vi "Call VI.vi"(4 "output info":T1[](array[typedef]), 6 "input info":T2[](array[typedef]), 8 "error in (no error)":errorcluster, 9 "Input Values":string[](array[string]), 10 "Input Names":string[](array[string]), 11 "VI in":refnum<vi>) -> (0 "error out":errorcluster, 1 "output values":string[](array[string]), 2 "output names":string[](array[string]), 3 "pictures":string[](array[string]))   [LabVIEW 2020, in "MCP Server.lvlib"]
uses:
  MCP Server.lvlib
  <vilib>/JDP Science/JSONtext/LVClass Serializer/JSONtext LVClass Serializer.lvclass
  e41d13a5-b533-4b14-93c6-4ba0c6d1a2bf.vi
  b3e15f38-d5ce-4610-9e48-04c139622bf1.vi
  b8448edb-b4b5-47d7-90b3-aea56ff88df2.vi
  989a8bd6-30de-4821-a40a-8a1d239f579d.vi
  8b9ff06f-0ef6-44a3-acf4-59db1b6b1b31.vi
  0616d323-15ae-486a-97f1-8f6250f713f5.vi
  9d91f7f2-9bb6-4ecb-af38-d838d0deb514.vi
  fd11c23e-f9de-4047-abc2-5cee66b205fd.vi
  1521ffbb-a9e1-42f7-9593-99dcb95d3f2d.vi
  522b1827-3836-432c-b8b2-8f0c55f6feb7.vi
  4168f984-ecba-4b3e-98aa-6b303e1fc845.vi
  4c506424-2eda-4aef-885b-07ff0af22ab5.vi
  543640a1-fb1b-49d2-854d-672a7e8b1deb.vi
  bf9e786f-d1ab-471f-a68b-f7992835e449.vi
  7e5c8ca1-4dad-4b78-a054-e5ecb6fe69da.vi
  804d9a9c-1e56-403f-8063-8c6c0e8f0982.vi
  Input Parameter.ctl
  Output Parameter.ctl
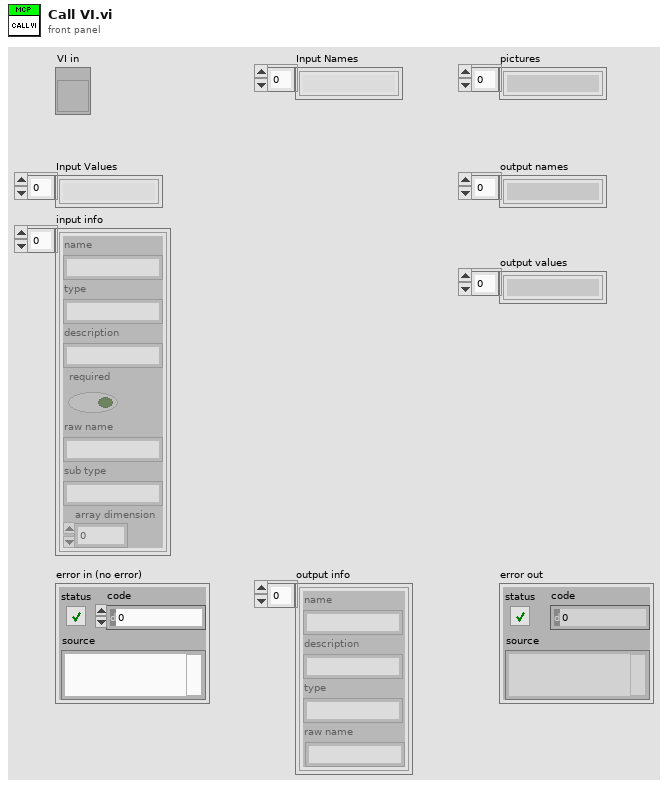
[diagram p1: front panel]
types:
  T1 = typedef "MCP Server.lvlib/Output Parameter.ctl" = cluster{"name":string, "description":string, "type":string, "raw name":string}
  T2 = typedef "MCP Server.lvlib/Input Parameter.ctl" = cluster{"name":string, "type":string, "description":string, "required":bool, "raw name":string, "sub type":string, "array dimension":i32}
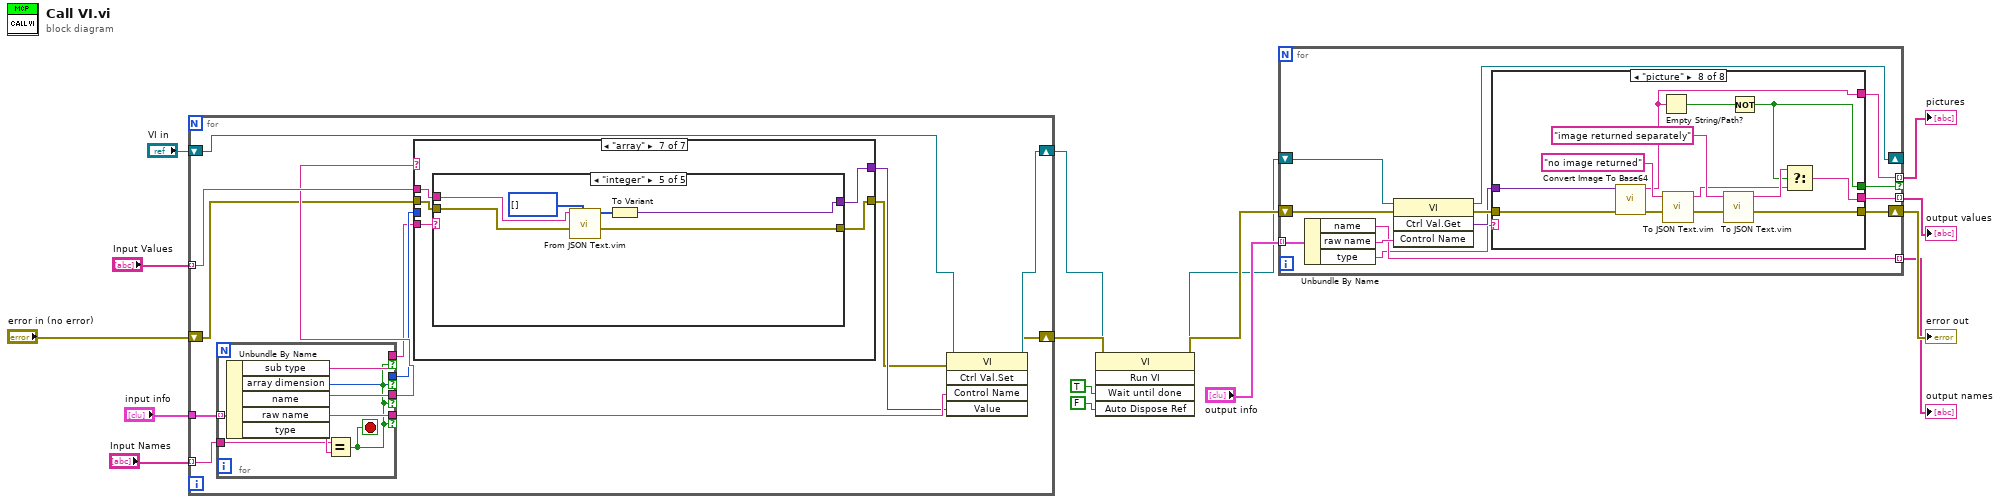
[diagram p0: block diagram]
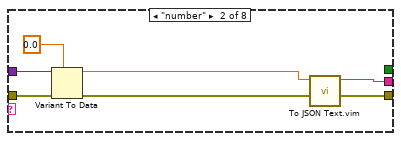
[diagram p3: hidden frame]
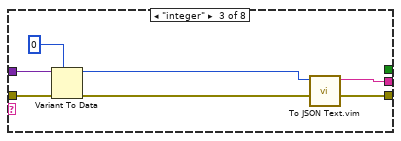
[diagram p4: hidden frame]
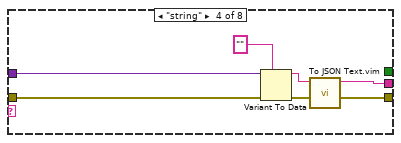
[diagram p5: hidden frame]
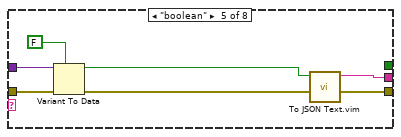
[diagram p6: hidden frame]
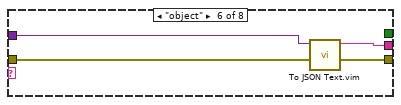
[diagram p7: hidden frame]
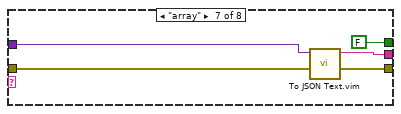
[diagram p8: hidden frame]
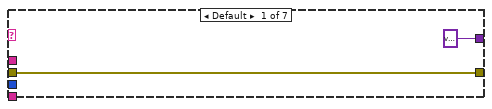
[diagram p9: hidden frame]
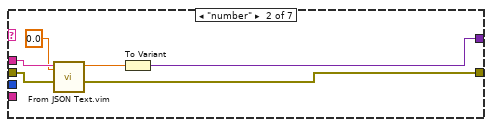
[diagram p10: hidden frame]
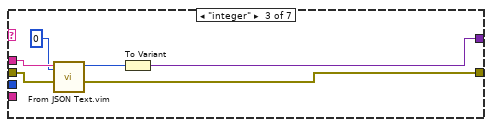
[diagram p11: hidden frame]
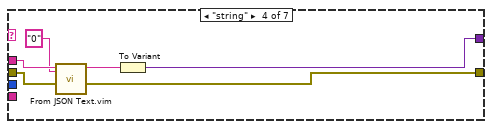
[diagram p12: hidden frame]
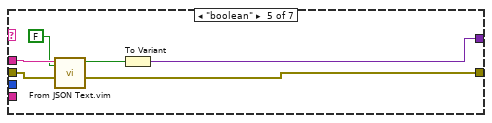
[diagram p13: hidden frame]
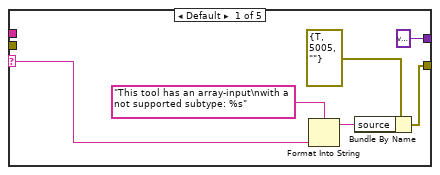
[diagram p15: hidden frame]
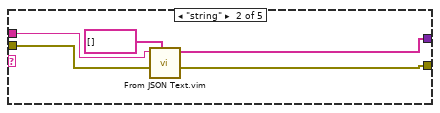
[diagram p16: hidden frame]
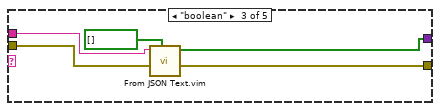
[diagram p17: hidden frame]
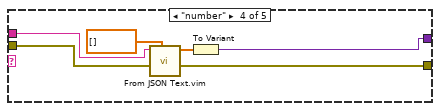
[diagram p18: hidden frame]
diagram:
  n1 = for {
    tunnel: "Input Values" -> [w23] mode=indexing
    tunnel: "Input Names" -> [w25] mode=indexing
    shift-right: [w28] -> w3
    shift-left: "VI in" -> [w29]
    shift-right: [w27] -> w4
    shift-left: "error in (no error)" -> [w20]
    tunnel: "input info" -> [w26]
    n2 = for {
      tunnel: w26 -> [w98] mode=indexing
      tunnel: w25 -> [w96]
      tunnel: [w95] -> w24 if=w91
      tunnel: [w94] -> w21 if=w91
      tunnel: [w93] -> w18 if=w91
      tunnel: [w92] -> w17 if=w91
      stop <- w91 stop-if-true
      n3 = Unbundle By Name(w98) -> ("sub type"=w92:string, "array dimension"=w93:i32, "name"=w97:string, "raw name"=w95:string, "type"=w94:string)
      n4 = Equal?(x=w96, y=w97) -> (x = y?=w91:bool)
    }
    n5 = case shown="\"array\"" w21 {
      tunnel: w23 -> [_ w37 w43 w49 w55 w57 w60]
      tunnel: [variant ("Variant") w35 w41 w47 w53 w57 w58] -> w22
      tunnel: w20 -> [w30 w33 w38 w45 w51 w56 w62]
      tunnel: [w30 w32 w39 w44 w50 w56 w61] -> w19
      tunnel: w18 -> [_ _ _ _ _ _ _]
      tunnel: w17 -> [_ _ _ _ _ _ w59]
      frame Default {
      }
      frame "number" {
        n6 = call "From JSON Text.vim"("Data Type and Default Value"=0.0, "error in (no error)"=w33, "JSON"=w37) -> ("error out"=w32:errorcluster, "Data out"=w36:dbl)  [unwired: 7 in]
        n7 = To Variant(anything=w36) -> (Variant=w35:variant)
      }
      frame "integer" {
        n8 = call "From JSON Text.vim"("Data Type and Default Value"=i64 0, "error in (no error)"=w38, "JSON"=w43) -> ("error out"=w39:errorcluster, "Data out"=w42:i64)  [unwired: 7 in]
        n9 = To Variant(anything=w42) -> (Variant=w41:variant)
      }
      frame "string" {
        n10 = call "From JSON Text.vim"("Data Type and Default Value"="0", "error in (no error)"=w45, "JSON"=w49) -> ("error out"=w44:errorcluster, "Data out"=w48:string)  [unwired: 7 in]
        n11 = To Variant(anything=w48) -> (Variant=w47:variant)
      }
      frame "boolean" {
        n12 = call "From JSON Text.vim"("Data Type and Default Value"=FALSE, "error in (no error)"=w51, "JSON"=w55) -> ("error out"=w50:errorcluster, "Data out"=w54:bool)  [unwired: 7 in]
        n13 = To Variant(anything=w54) -> (Variant=w53:variant)
      }
      frame "object" {
      }
      frame "array" {
        n14 = case shown="\"integer\"" w59 {
          selector: w59 -> [w64 _ _ _ _]
          tunnel: w62 -> [_ w73 w78 w84 w90]
          tunnel: [w67 w72 w77 w83 w89] -> w61
          tunnel: w60 -> [_ w71 w76 w82 w88]
          tunnel: [variant ("Variant") w69 w74 w79 w85] -> w58
          frame Default {
            n15 = Format Into String(format string="This tool has an array-input\nwith a not supported subtype: %s" ("source"), w64) -> (resulting string=w65:string)  [unwired: 2 in, 1 out]
            n16 = Bundle By Name(cluster=errorcluster {"status"=TRUE, "code"=5005, "source"=""} ("error out"), "source"=w65) -> (w67:errorcluster)
          }
          frame "string" {
            n17 = call "From JSON Text.vim"("Data Type and Default Value"=string[] [] ("Input Values"), "error in (no error)"=w73, "JSON"=w71) -> ("error out"=w72:errorcluster, "Data out"=w69:string[])  [unwired: 7 in]
          }
          frame "boolean" {
            n18 = call "From JSON Text.vim"("Data Type and Default Value"=bool[] [] ("Input Values"), "error in (no error)"=w78, "JSON"=w76) -> ("error out"=w77:errorcluster, "Data out"=w74:bool[])  [unwired: 7 in]
          }
          frame "number" {
            n19 = call "From JSON Text.vim"("Data Type and Default Value"=dbl[] [] ("Input Values"), "error in (no error)"=w84, "JSON"=w82) -> ("error out"=w83:errorcluster, "Data out"=w80:dbl[])  [unwired: 7 in]
            n20 = To Variant(anything=w80) -> (Variant=w79:variant)
          }
          frame "integer" {
            n21 = call "From JSON Text.vim"("Data Type and Default Value"=i64[] [] ("Input Values"), "error in (no error)"=w90, "JSON"=w88) -> ("error out"=w89:errorcluster, "Data out"=w86:i64[])  [unwired: 7 in]
            n22 = To Variant(anything=w86) -> (Variant=w85:variant)
          }
        }
      }
    }
    n23 = invoke class="VI" method="Ctrl Val.Set"(reference=w29, error in=w19, "Control Name"=w24, "Value"=w22) -> (reference out=w28:refnum<vi>, error out=w27:errorcluster)  [unwired: 1 in, 3 out]
  }
  n24 = invoke class="VI" method="Run VI"(reference=w3, error in=w4, "Wait until done"=TRUE ("Wait Until Done"), "Auto Dispose Ref"=FALSE ("Auto Dispose Reference")) -> (reference out=w7:refnum<vi>, error out=w8:errorcluster)  [unwired: 1 in, 3 out]
  n25 = for {
    shift-right: [w110] -> _
    shift-left: w7 -> [w111]
    shift-right: [w103] -> w15
    shift-left: w8 -> [w108]
    tunnel: "output info" -> [w107] mode=indexing
    tunnel: [w104] -> w11 mode=indexing
    tunnel: [w102] -> w10 mode=indexing
    tunnel: [w100] -> w13 mode=indexing if=w99
    n26 = Unbundle By Name(w107) -> ("name"=w104:string, "raw name"=w105:string, "type"=w101:string)
    n27 = invoke class="VI" method="Ctrl Val.Get"(reference=w111, error in=w108, "Control Name"=w105) -> (reference out=w110:refnum<vi>, error out=w109:errorcluster, "Get Control Value Variant"=w106:variant)  [unwired: 1 in, 1 out]
    n28 = case shown="\"picture\"" w101 {
      tunnel: w109 -> [w112 w119 w126 w133 w140 w144 w149 w161]
      tunnel: w106 -> [_ w115 w122 w129 w136 w141 w145 w162]
      tunnel: [w112 w118 w125 w132 w139 w143 w148 w158] -> w103
      tunnel: [_ w117 w124 w131 w138 w142 w146 w155] -> w102
      tunnel: [_ _ _ _ _ _ _ w156] -> w100
      tunnel: [_ _ _ _ _ _ FALSE w152] -> w99
      frame Default {
      }
      frame "number" {
        n29 = Variant To Data(error in=w119, type=0.0, Variant=w115) -> (data=w113:dbl, error out=w116:errorcluster)
        n30 = call "To JSON Text.vim"("error in (no error)"=w116, "Anything"=w113) -> ("error out"=w118:errorcluster, "<JSON>"=w117:string)  [unwired: 8 in]
      }
      frame "integer" {
        n31 = Variant To Data(error in=w126, type=i64 0, Variant=w122) -> (data=w120:i64, error out=w123:errorcluster)
        n32 = call "To JSON Text.vim"("error in (no error)"=w123, "Anything"=w120) -> ("error out"=w125:errorcluster, "<JSON>"=w124:string)  [unwired: 8 in]
      }
      frame "string" {
        n33 = Variant To Data(error in=w133, type="", Variant=w129) -> (data=w127:string, error out=w130:errorcluster)
        n34 = call "To JSON Text.vim"("error in (no error)"=w130, "Anything"=w127) -> ("error out"=w132:errorcluster, "<JSON>"=w131:string)  [unwired: 8 in]
      }
      frame "boolean" {
        n35 = Variant To Data(error in=w140, type=FALSE, Variant=w136) -> (data=w134:bool, error out=w137:errorcluster)
        n36 = call "To JSON Text.vim"("error in (no error)"=w137, "Anything"=w134) -> ("error out"=w139:errorcluster, "<JSON>"=w138:string)  [unwired: 8 in]
      }
      frame "object" {
        n37 = call "To JSON Text.vim"("error in (no error)"=w144, "Anything"=w141) -> ("error out"=w143:errorcluster, "<JSON>"=w142:string)  [unwired: 8 in]
      }
      frame "array" {
        n38 = call "To JSON Text.vim"("error in (no error)"=w149, "Anything"=w145) -> ("error out"=w148:errorcluster, "<JSON>"=w146:string)  [unwired: 8 in]
      }
      frame "picture" {
        n39 = call "Convert Image To Base64.vi"("error in (no error)"=w161, "Get Control Value Variant"=w162) -> ("error out"=w151:errorcluster, "<JSON>"=w156:string)  [unwired: 8 in]
        n40 = Empty String/Path?(string/path=w156) -> (empty?=w153:bool)
        n41 = call "To JSON Text.vim"("error in (no error)"=w151, "Anything"="no image returned" ("<JSON>")) -> ("error out"=w150:errorcluster, "<JSON>"=w154:string)  [unwired: 8 in]
        n42 = call "To JSON Text.vim"("error in (no error)"=w150, "Anything"="image returned separately" ("<JSON>")) -> ("error out"=w158:errorcluster, "<JSON>"=w159:string)  [unwired: 8 in]
        n43 = Not(x=w153) -> (.not. x?=w152:bool)
        n44 = Select(t=w159, s=w152, f=w154) -> (s? t:f=w155:string)
      }
    }
  }
  "error out" <- w15
  "pictures" <- w13
  "output names" <- w11
  "output values" <- w10
